vi "GetValueForKey.vi"() -> ()   [LabVIEW 2018]
panel:
  in  "Key":string="everything"
  in  "Dictionary":cluster{"Key":string, "value":dbl}[](array[cluster])=[{"Key"="test", "value"=123.0}, {"Key"="test2", "value"=456.0}, {"Key"="everything", "value"=42.0}]
  out "value":dbl
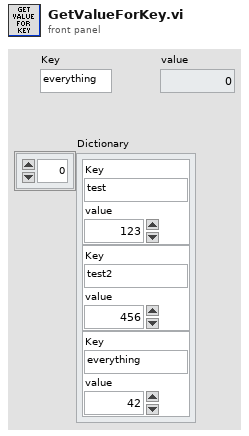
[diagram p1: front panel]
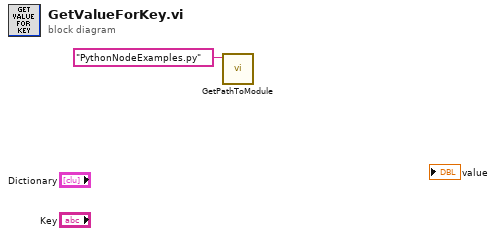
[diagram p0: block diagram]
diagram:
  n1 = call "GetPathToModule.vi"("module name"="PythonNodeExamples.py") -> ()  [unwired: 10 in, 1 out]
